vi "Reconfig Local Module.vi"(8 "error in (no error)":errorcluster, 9 "Config Channels":dbl[](array[numeric]), 10 "IOV ref":refnum<k21>, 11 "Module DVR":refnum<data-value>) -> (0 "error out":errorcluster)   [LabVIEW 2027, in "SEECD Engine.lvlib"]
uses:
  SEECD Engine.lvlib
  Includes/Modules.lvlibp/RSI Module/RSI Module.lvclass
  <vilib>/NI VeriStand/Custom Device Tools/Custom Device Utility Library/Custom Device Utility Library.lvlib
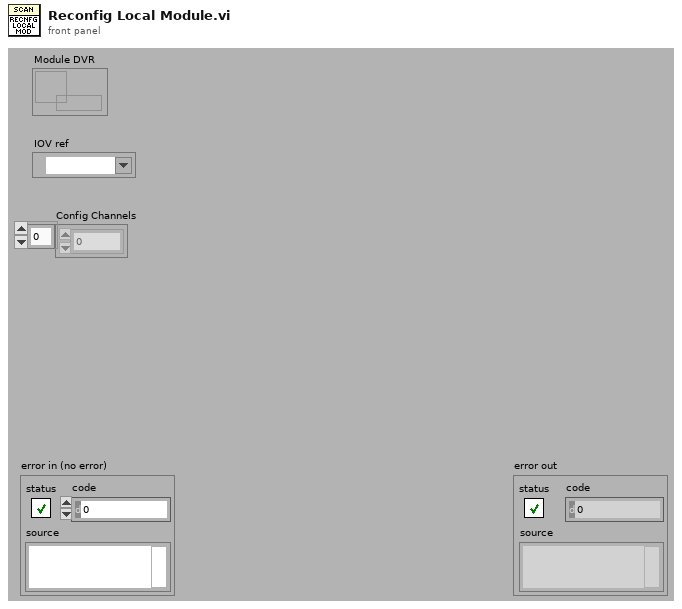
[diagram p1: front panel]
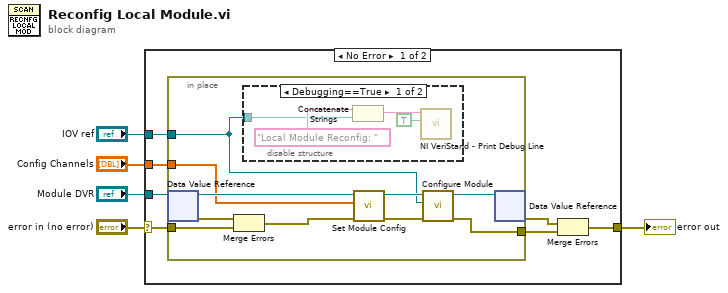
[diagram p0: block diagram]
diagram:
  n1 = case shown="No Error" "error in (no error)" {
    selector: "error in (no error)" -> [w11 w27]
    tunnel: [w6 w27] -> w4
    tunnel: "Module DVR" -> [w12 _]
    tunnel: "Config Channels" -> [w10 _]
    tunnel: "IOV ref" -> [w9 _]
    frame No Error {
      n2 = in-place {
        in-place-border: w11 -> [w21]
        in-place-border: w10 -> [w18]
        in-place-border: w9 -> [w13]
        in-place-border: [w14] -> w7
        n3 = in-place-dvr #1(w12) -> (w19:refnum<class "RSI Module.lvclass">, w22:errorcluster)
        n4 = Merge Errors(w22, w21) -> (w20:errorcluster)
        n5 = disable-structure shown="Debugging==True" {
          disable-tunnel: w13 -> [w24 _]
          frame condition #0 {
            n6 = Concatenate Strings("Local Module Reconfig: " ("string"), w24) -> (w26:string)
            n7 = call <vilib>:"NI VeriStand - Print Debug Line.vi"("Add to log file? (F)"=TRUE, "Message"=w26) -> ()  [unwired: 9 in, 1 out]
          }
          frame condition #1 (active) {
          }
        }
        n8 = call-dynamic "Set Module Config.vi"("error in (no error)"=w20, "Config Channels"=w18, "RSI Module in"=w19) -> ("error out"=w17:errorcluster, "RSI Module out"=w16:refnum<class "RSI Module.lvclass">)  [unwired: 7 in]
        n9 = call-dynamic "Configure Module.vi"("error in (no error)"=w17, "IOV ref in"=w13, "RSI Module in"=w16) -> ("error out"=w14:errorcluster, "RSI Module out"=w15:refnum<class "RSI Module.lvclass">)  [unwired: 6 in, 1 out]
        n10 = in-place-dvr #1(w15) -> (w8:errorcluster)  [unwired: 1 out]
      }
      n11 = Merge Errors(w8, w7) -> (w6:errorcluster)
    }
    frame Error {
    }
  }
  "error out" <- w4
